vi "timeline_config.vi"() -> ()   [LabVIEW 2026]
uses:
  <vilib>/addons/_JKI.lib/Serialization/JSON/JKI JSON Serialization.lvlib
panel:
  in  "Number of Days":dbl=5.0
  in  "?":bool
  out "Preview":string
  in  "Clear / Reset":bool
  in  "Generate JSON":bool
  out "Status Message":string
  in  "Save Path":path
  in  "Days Array":T1(array[cluster])
  # "Actions"
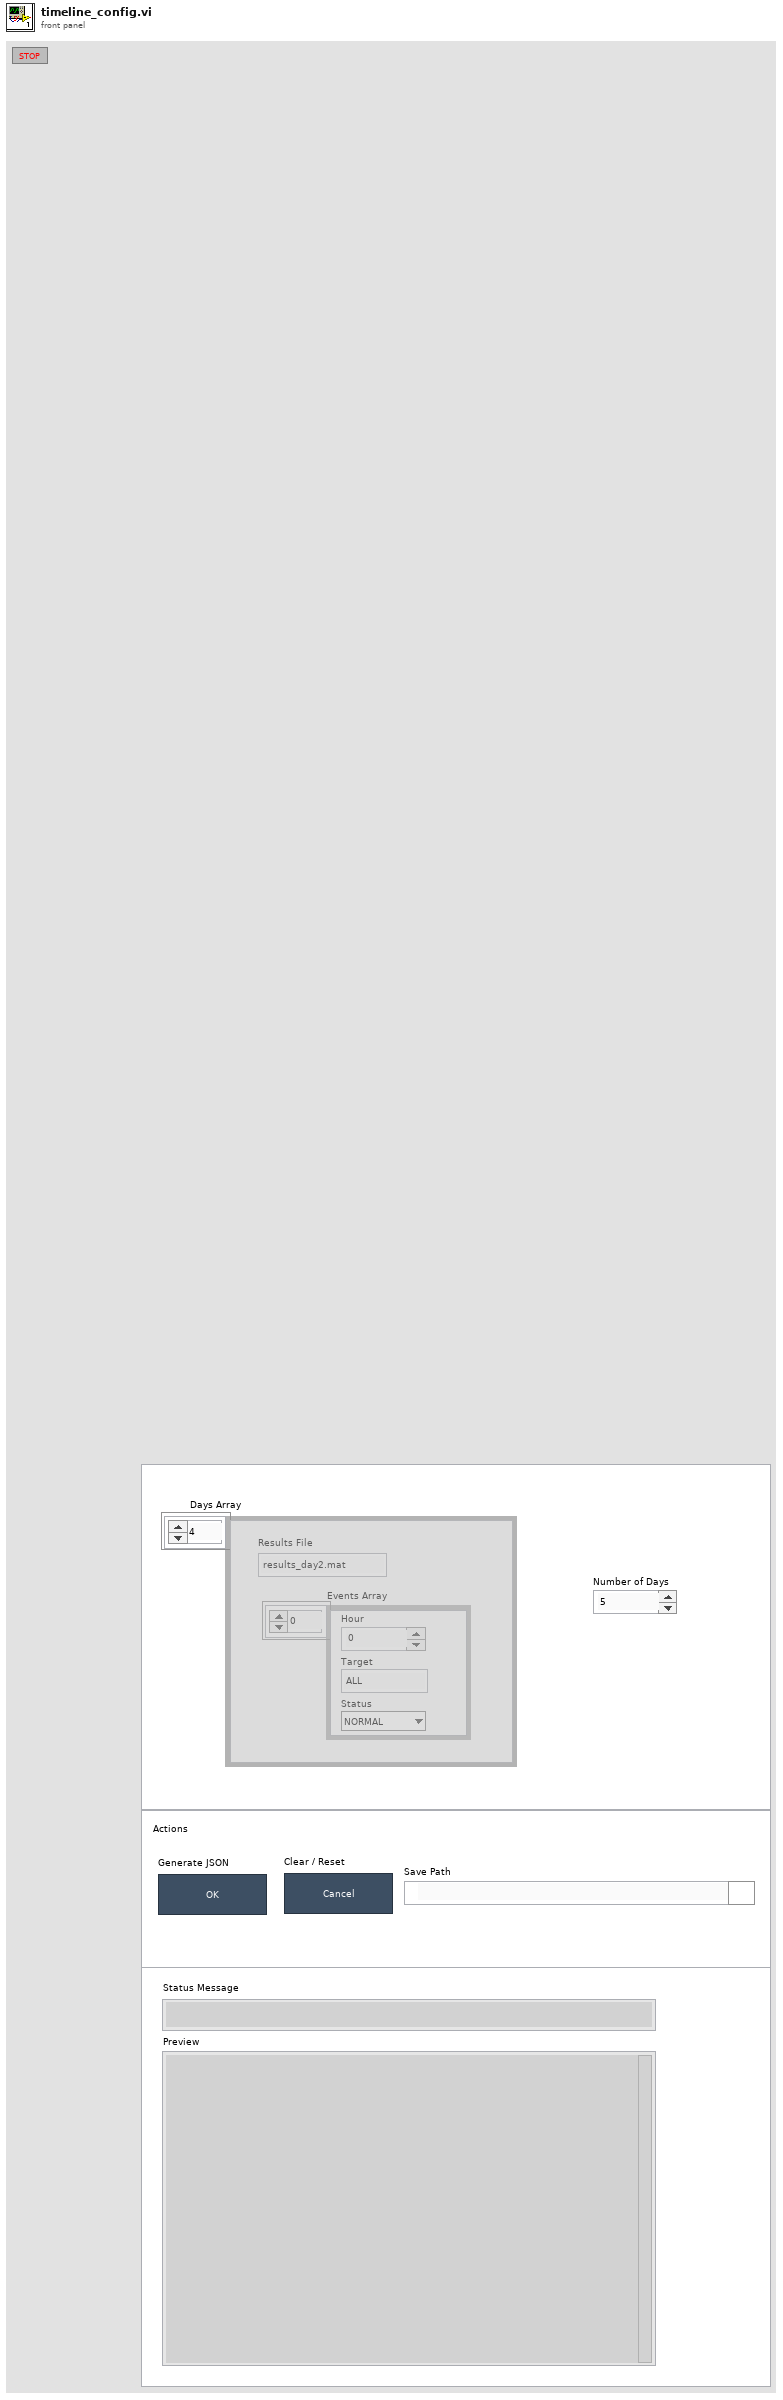
[diagram p1: front panel]
types:
  T1 = cluster{"results_file":string, "events":cluster{"hour":dbl, "target":string, "status":enum16{"", "NORMAL", "OFFLINE", "FAULTED", "SHED", "WARNING"}}[]}[]
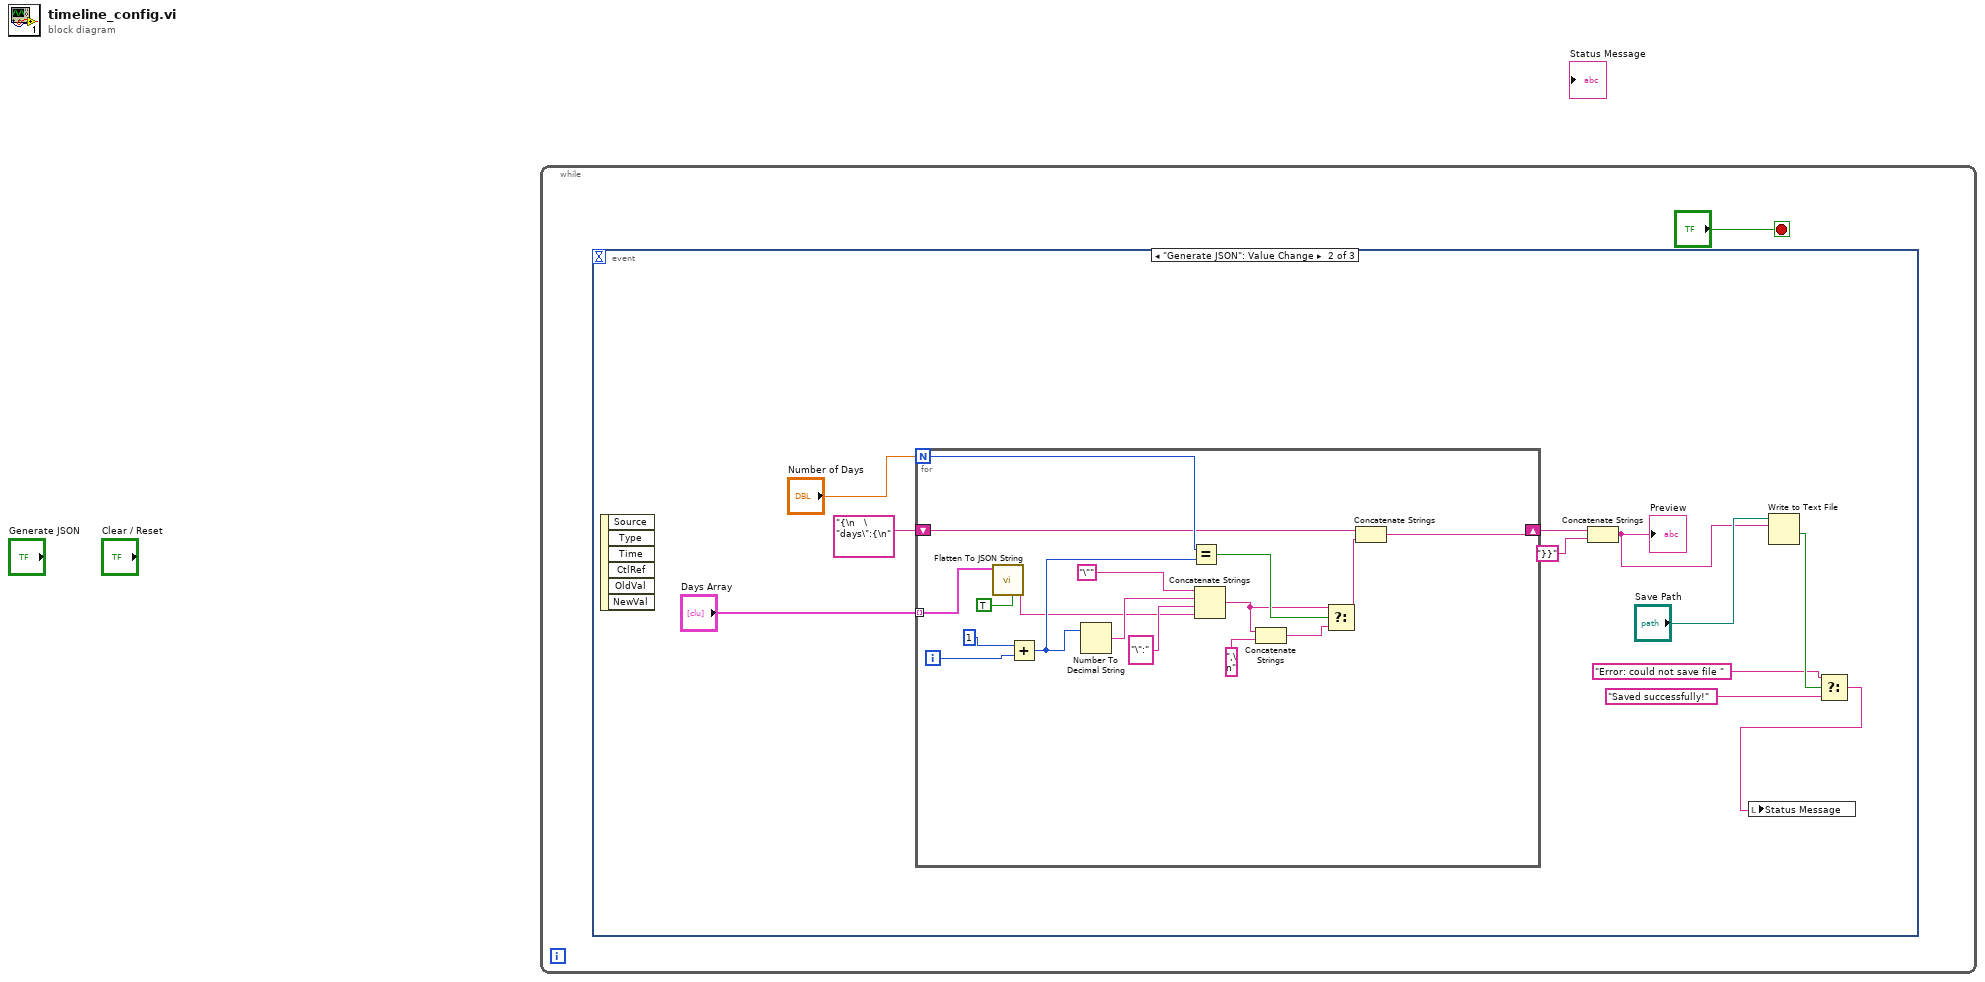
[diagram p0: block diagram]
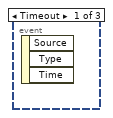
[diagram p2: hidden frame]
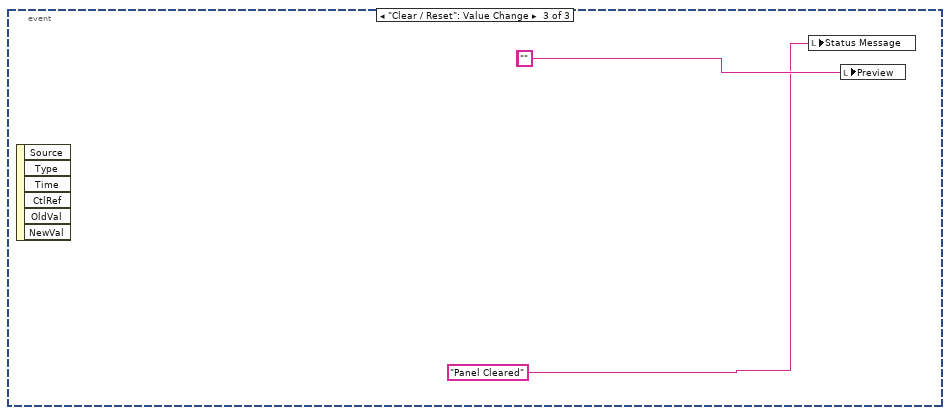
[diagram p3: hidden frame]
diagram:
  n1 = while {
    stop <- "?" stop-if-true
    n2 = event shown="[1] \"Generate JSON\": Value Change" {
      selector: _ -> [_ _ _]
      dyn-events: _ -> [_ _ _]
      timeout: _ -> [_ _ _]
      event Timeout {
        n3 = event-data() -> ()  [unwired: 1 in, 3 out]
      }
      event "Generate JSON": Value Change {
        n4 = event-data() -> ()  [unwired: 1 in, 6 out]
        n5 = for {
          N: "Number of Days" -> [w25]
          tunnel: "Days Array" -> [w13] mode=indexing
          shift-right: [w18] -> w10
          shift-left: "{\n   \"days\":{\n" -> [w20]
          i -> [w29]
          n6 = call <vilib>:"Flatten To JSON String.vi"("Enums As String (F)"=TRUE, "Variant"=w13) -> ("JSON String"=w15:string)  [unwired: 8 in, 1 out]
          n7 = Add(x=1, y=w29) -> (x+y=w26:i32)
          n8 = Number To Decimal String(number=w26) -> (decimal integer string=w17:string)  [unwired: 1 in]
          n9 = Equal?(x=w25, y=w26) -> (x = y?=w23:bool)
          n10 = Concatenate Strings("\"", w17, "\":", w15) -> (w22:string)
          n11 = Concatenate Strings(w22, ",\n") -> (w21:string)
          n12 = Select(t=w22, s=w23, f=w21) -> (s? t:f=w19:string)
          n13 = Concatenate Strings(w20, w19) -> (w18:string)
        }
        n14 = Concatenate Strings(w10, "}}") -> (w3:string)
        "Preview" <- w3
        n15 = Write to Text File(file (use dialog)="Save Path", text=w3) -> (cancelled=w7:bool)  [unwired: 2 in, 2 out]
        n16 = Select(t="Error: could not save file ", s=w7, f="Saved successfully!") -> (s? t:f=w2:string)
        n17 = local write "Status Message"(w2) -> ()
      }
      event "Clear / Reset": Value Change {
        (unwired) ""
        n18 = event-data() -> ()  [unwired: 1 in, 6 out]
        n19 = local write "Status Message"("Panel Cleared") -> ()
        n20 = local write "Preview"("") -> ()
      }
    }
  }
